vi "Main Editor UI.vi"() -> ()   [LabVIEW 2015, in "J1939 editor node.lvclass"]
doc: "This is the main view for configuration the behavior of a module in the DCAF standard editor."
uses:
  J1939 editor node.lvclass
  <vilib>/NI/Configuration Framework/Node/NodeRef.ctl
  <vilib>/NI/Configuration Framework/Node/NISE_CEF_Node.lvclass
  <vilib>/NI/AMC/Message Queue.ctl
  <vilib>/NI/AMC/Message.ctl
  <vilib>/NI/Tools/Keyed Array/KeyedArray.ctl
  <vilib>/NI/Configuration Framework/Node/UserEventRef.ctl
  <vilib>/NI/Configuration Framework/Controls/EventCluster.ctl
  <vilib>/NI/DCAF UI Toolkit/Controls/Configure.ctl
  <vilib>/NI/DCAF UI Toolkit/Controls/Add.ctl
  <vilib>/NI/DCAF UI Toolkit/Controls/Remove.ctl
  <vilib>/NI/Configuration Framework/Node/StopEvent.ctl
  <vilib>/NI/Configuration Framework/Node/RefreshUIEvent.ctl
  <vilib>/NI/Configuration Framework/Node/CacheState.ctl
  <vilib>/NI/Configuration Framework/Node/NodeChangeEvent.ctl
  <vilib>/NI/Tag Bus/tag/Data Type.ctl
  Permissions Enum.ctl
  <vilib>/NI/DCAF/Tag Editor Core/Table API/Available Tag Menu/channel action event.ctl
  <vilib>/NI/DCAF/Tag Editor Core/Table API/Available Tag Menu/dialog output action.ctl
  <vilib>/NI/Tag Bus Module Framework/channel/TBM channel.lvclass
  <vilib>/NI/Tag Bus/tag/tag descriptor.lvclass
  <vilib>/NI/DCAF/Tag Editor Core/Table API/Table Manager/Call Back Ref Type Def.ctl
  <vilib>/NI/DCAF/Tag Editor Core/Configuration Editor/Classes/Engine Parent/Engine Parent Editor Node.lvclass
  <vilib>/NI/DCAF/Tag Editor Core/Configuration Editor/Classes/Module editor node/module editor node.lvclass
  module/configuration/XNET Settings.ctl
  <vilib>/NI/DCAF/Tag Editor Core/Table API/Table Manager/references.ctl
  <vilib>/Utility/miscctls.llb/LVPositionTypeDef.ctl
  <vilib>/NI/DCAF/Tag Editor Core/Table API/Listbox/Multi Column Listbox.lvclass
  <vilib>/NI/Configuration Framework/NISE_CEF_TreeControl.lvlib
  <vilib>/NI/Tools/Keyed Array/Tools_KeyedArray.lvlib
  <vilib>/NI/AMC/AMC.lvlib
  <vilib>/NI/DCAF/Tag Editor Core/Table API/Table Manager.lvlib
  <vilib>/NI/DCAF/Tag Editor Core/Table API/Table Manager/Table Manager.lvclass
  <vilib>/NI/DCAF UI Toolkit/Controls/DCAF UI Elements.lvlib
  module/configuration/J1939 configuration.lvclass
panel:
  in  "user event out":refnum<user-event>
  in  "Permissions":T1
  in  "data type":T2
  in  "node change":T3
  in  "cache state":T4
  in  "refresh UI":T5
  in  "stop event":T6
  in  "Tab Control":enum32{"Channels", "XNET Settings"}(tab)
  in  "Remove Button":T7
  in  "Add Button":T8
  in  "Table":i32(listbox)
  in  "settings":T9
  in  "XNET Settings":T10={"Select Interface"="CAN2", "Claim By Adress"=FALSE, "Node Address"=1, "Node Name"=1}
  in  "user event":T11
  in  "main queue":T12
  in  "node ref":T13
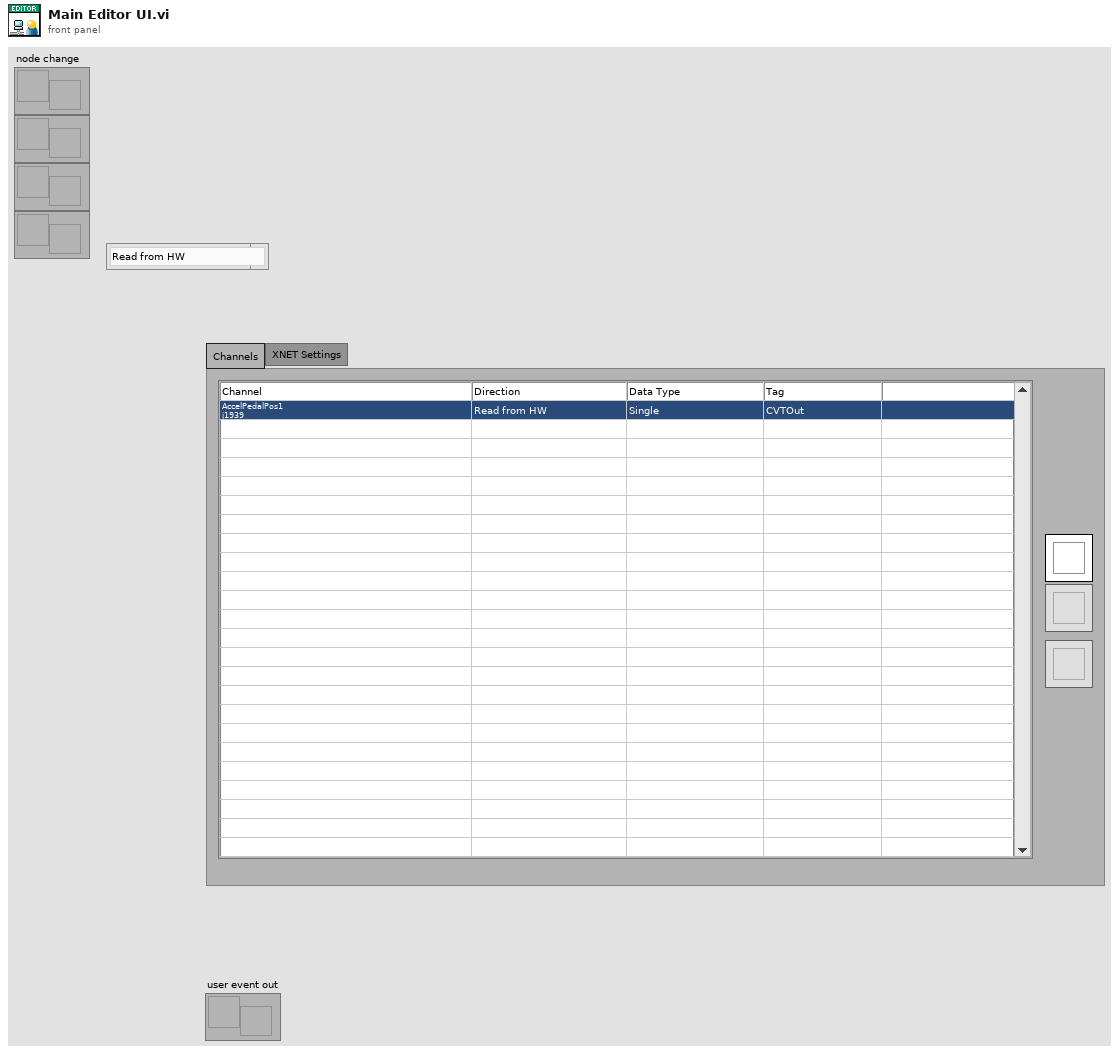
[diagram p1: front panel]
types:
  T1 = typedef "J1939 editor node.lvclass/Permissions Enum.ctl" = enum16{"Read from HW", "Write to HW"}
  T2 = typedef "tag bus.lvlib/tag descriptor.lvclass/Data Type.ctl" = enum16{"Double", "Single", "I64", "I32", "I16", "I8", "U64", "U32", "U16", "U8", "Boolean", "String", "Array of Double", "Array of Single", "Array of I64", "Array of I32", "Array of I16", "Array of I8", "Array of U64", "Array of U32", "Array of U16", "Array of U8", "Array of Boolean", "Array of String"}
  T3 = typedef "NISE_CEF_Node.lvclass/NodeChangeEvent.ctl" = refnum<user-event>
  T4 = typedef "NISE_CEF_Node.lvclass/CacheState.ctl" = refnum<user-event>
  T5 = typedef "NISE_CEF_Node.lvclass/RefreshUIEvent.ctl" = refnum<user-event>
  T6 = typedef "NISE_CEF_Node.lvclass/StopEvent.ctl" = refnum<user-event>
  T7 = typedef "DCAF UI Elements.lvlib/Remove.ctl" = bool
  T8 = typedef "DCAF UI Elements.lvlib/Add.ctl" = bool
  T9 = typedef "DCAF UI Elements.lvlib/Configure.ctl" = bool
  T10 = typedef "J1939 configuration.lvclass/XNET Settings.ctl" = cluster{"Select Interface":refnum<k21>, "Claim By Adress":bool, "Node Address":u8, "Node Name":u64}
  T11 = typedef "NISE_CEF_Node.lvclass/UserEventRef.ctl" = refnum<user-event>
  T12 = typedef "AMC.lvlib/Message Queue.ctl" = refnum<queue>
  T13 = typedef "NISE_CEF_Node.lvclass/NodeRef.ctl" = refnum<data-value>
  T14 = typedef "Table Manager.lvlib/Table Manager.lvclass/references.ctl" = cluster{"stop event":T6, "refresh UI":T5, "cache state":T4, "node change":T3, "user event out":refnum<user-event>, "main queue":T12, "user event":T11}
  T15 = typedef "LVPositionTypeDef.ctl" = cluster{"Left":i32, "Top":i32}
  T16 = typedef "Table Manager.lvlib/Table Manager.lvclass/object ref.ctl" = cluster{"engine":refnum<data-value>, "Node Ref":refnum<data-value>}
  T17 = typedef "Table Manager.lvlib/Column.lvclass/Column Descriptor.ctl" = cluster{"name":string, "caption":string, "Column Type":T18, "Params":string, "AutoSizeMode":i32, "FillWeight":sgl, "MinWidth":u32, "tooltip":string, "Enum Reference":refnum<vi>, "Channel suffix":string, "Read Only":bool, "Call Back VI":T19, "DT Dependency":i32, "name dependency":i32, "data type":T2, "Custom Column":refnum<class "Column.lvclass">}
  T18 = typedef "Table Manager.lvlib/Column.lvclass/Column Type.ctl" = enum16{"String", "Mapping", "Enum", "Custom"}
  T19 = typedef "Table Manager.lvlib/Table Manager.lvclass/Call Back Ref Type Def.ctl" = refnum<vi>
  T20 = typedef "Table Manager.lvlib/Table Manager.lvclass/Table Events.ctl" = cluster{"Menu Selection":refnum<user-event>}
  T21 = enum8{"Enabled", "Disabled", "Disabled and Grayed Out"}
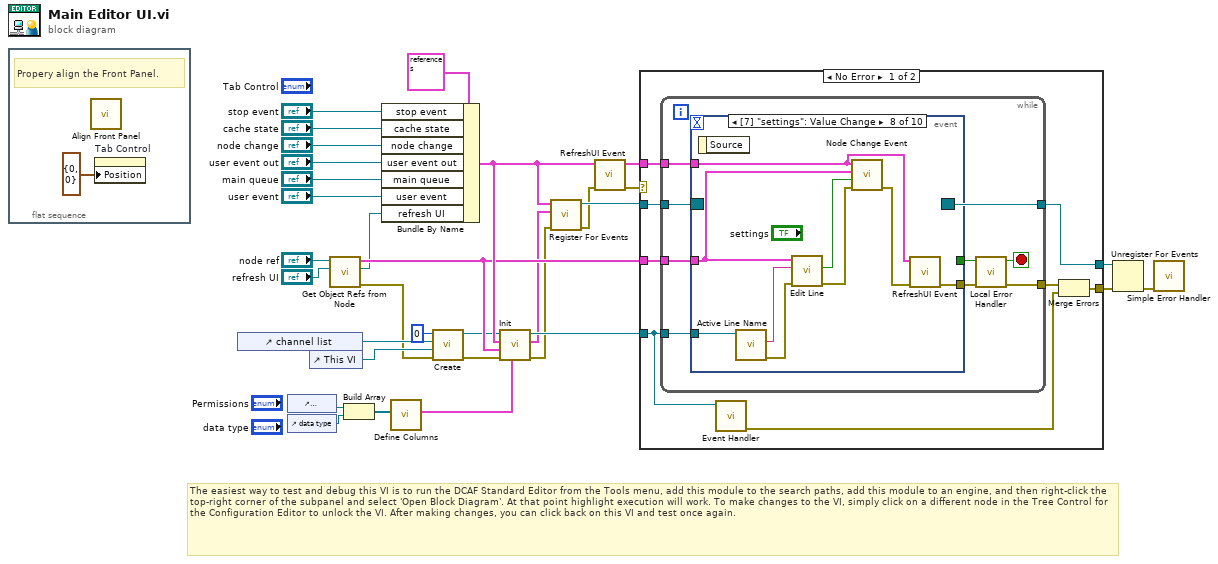
[diagram p0: block diagram]
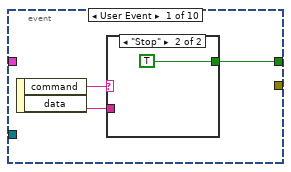
[diagram p2: hidden frame]
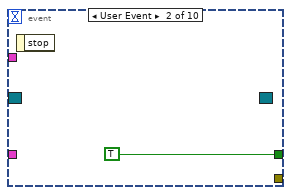
[diagram p4: hidden frame]
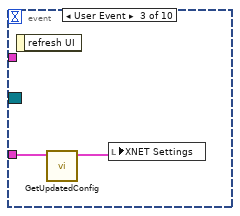
[diagram p5: hidden frame]
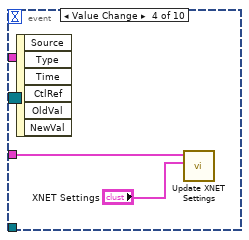
[diagram p6: hidden frame]
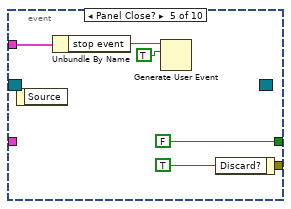
[diagram p7: hidden frame]
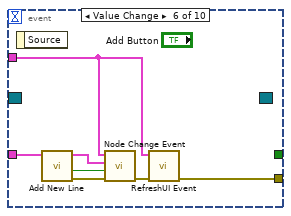
[diagram p8: hidden frame]
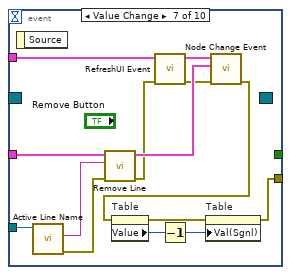
[diagram p9: hidden frame]
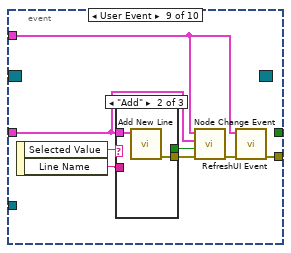
[diagram p10: hidden frame]
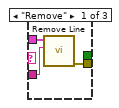
[diagram p11: hidden frame]
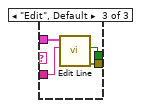
[diagram p12: hidden frame]
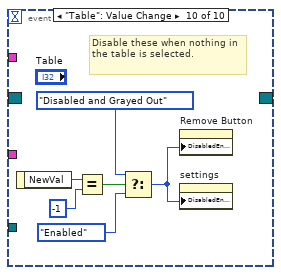
[diagram p13: hidden frame]
diagram:
  # "The easiest way to test and debug this VI is to run the DCAF Standard Editor from the Tools menu, add this module to the search paths, add this module to an engine, and then right-click the top-right corner of the subpanel and select 'Open Block Diagram'. At that point highlight execution will work. To make changes to the VI, simply click on a different node in the Tree Control for the Configuration Editor to unlock the VI. After making changes, you can click back on this VI and test once again."
  n1 = flat-sequence {
    frame #0 {
      # "Propery align the Front Panel."
      n2 = call <vilib>:"Align Front Panel.vi"() -> ()  [unwired: 10 in, 2 out]
      n3 = property on="Tab Control" class="TabCtl (strict)"("Position"=T15 {"Left"=0, "Top"=0}) -> ()  [unwired: 2 in, 2 out]
    }
  }
  n4 = control-ref of="channel list"() -> (w8:refnum<vi>)
  n5 = control-ref of="Permissions"() -> (w18:refnum<vi>)
  n6 = control-ref of="data type"() -> (w17:refnum<vi>)
  n7 = control-ref of="This VI"() -> (w6:refnum<vi>)
  n8 = call "Get Object Refs from Node.vi"("Refresh UI"="refresh UI", "Data Value Reference in"="node ref") -> ("error out"=w3:errorcluster, "Refresh UI out"=w1:T5, "References"=w15:T16)  [unwired: 7 in]
  n9 = Build Array(w18, w17) -> (w16:refnum<vi>[])
  n10 = Bundle By Name(cluster=T14 {"stop event"=refnum, "refresh UI"=refnum, "cache state"=refnum, "node change"=refnum, "user event out"=refnum, "main queue"=refnum, "user event"=refnum} ("References"), "stop event"="stop event", "cache state"="cache state", "node change"="node change", "user event out"="user event out", "main queue"="main queue", "user event"="user event", "refresh UI"=w1) -> (w19:T14)
  n11 = call "Define Columns.vi"("Enum Array"=w16) -> ("Column Definition"=w21:T17[])  [unwired: 10 in]
  n12 = call <vilib>:"Create.vi"("error in (no error)"=w3, "Top VI"=w6, "Listbox"=w8, "Index"=0) -> ("error out"=w4:errorcluster, "reference out"=w5:refnum<class "Multi Column Listbox.lvclass">)  [unwired: 6 in]
  n13 = call-dynamic "Init.vi"("Column Descriptors"=w21, "error in (no error)"=w4, "Node object refs"=w15, "Event References"=w19, "Multi Column Listbox in"=w5) -> ("error out"=w10:errorcluster, "Table Events"=w9:T20, "Multi Column Listbox out"=w14:refnum<class "Multi Column Listbox.lvclass">)  [unwired: 4 in]
  n14 = call "Register For Events.vi"("error in"=w10, "Table Events"=w9, "References"=w19) -> ("error out"=w12:errorcluster, "Event Registration Refnum"=w22:refnum<event-registration>)  [unwired: 7 in]
  n15 = call "RefreshUI Event.vi"("error in (no error)"=w12, "References in"=w19) -> ("error out"=w11:errorcluster, "References out"=w20:T14)  [unwired: 8 in]
  n16 = case shown="No Error" w11 {
    selector: w11 -> [_ w117]
    tunnel: w22 -> [w41 w116]
    tunnel: [w40 w116] -> w32
    tunnel: [w34 w117] -> w31
    tunnel: w20 -> [w39 _]
    tunnel: w15 -> [w38 _]
    tunnel: w14 -> [w37 _]
    frame No Error {
      n17 = while {
        tunnel: w41 -> [w50]
        tunnel: [w49] -> w40
        tunnel: [w46] -> w35
        tunnel: w39 -> [w44]
        tunnel: w38 -> [w43]
        tunnel: w37 -> [w42]
        stop <- w48 stop-if-true
        n18 = event shown="[7] \"settings\": Value Change" {
          selector: w50 -> [_ _ _ _ _ _ _ _ _ _]
          dyn-events: [_ _ _ _ _ _ _ _ _ _] -> w49
          timeout: _ -> [_ _ _ _ _ _ _ _ _ _]
          tunnel: [w53 TRUE _ _ FALSE _ _ _ _ _] -> w47
          tunnel: [_ _ _ _ _ w65 w72 w86 w98 _] -> w45
          tunnel: w44 -> [_ _ _ _ w61 w69 w83 w84 w94 _]
          tunnel: w43 -> [_ _ w57 w59 _ w70 w82 w90 w95 _]
          tunnel: w42 -> [_ _ _ _ _ _ w78 w91 _ _]
          event User Event {
            n19 = event-data() -> ("command"=w52:string, "data"=w51:string)  [unwired: 1 in]
            n20 = case shown="\"Stop\"" w52 {
              tunnel: [_ TRUE] -> w53
              tunnel: w51 -> [_ _]
              frame Default {
              }
              frame "Stop" {
              }
            }
          }
          event User Event {
            n21 = event-data() -> ()  [unwired: 1 in, 1 out]
          }
          event User Event {
            n22 = event-data() -> ()  [unwired: 1 in, 1 out]
            n23 = call "GetUpdatedConfig.vi"("References"=w57) -> ("XNET Settings"=w56:T10)  [unwired: 10 in]
            n24 = local write "XNET Settings"(w56) -> ()
          }
          event Value Change {
            n25 = event-data() -> ()  [unwired: 1 in, 6 out]
            n26 = call "Update XNET Settings.vi"("XNET Settings"="XNET Settings", "References"=w59) -> ()  [unwired: 10 in]
          }
          event Panel Close? {
            n27 = event-data() -> ()  [unwired: 1 in, 1 out]
            n28 = Unbundle By Name(w61) -> ("stop event"=w60:T6)
            n29 = Generate User Event(user event=w60, event data cluster=TRUE ("event data")) -> ()  [unwired: 2 in, 2 out]
            n30 = event-data("Discard?"=TRUE) -> ()  [unwired: 1 in, 1 out]
          }
          event Value Change {
            n31 = event-data() -> ()  [unwired: 1 in, 1 out]
            n32 = call "Add New Line.vi"("objects"=w70) -> ("error out"=w68:errorcluster, "success"=w66:bool)  [unwired: 8 in, 1 out]
            n33 = call "Node Change Event.vi"("error in (no error)"=w68, "Send (T)"=w66, "objects"=w70, "References in"=w69) -> ("error out"=w67:errorcluster)  [unwired: 7 in]
            n34 = call "RefreshUI Event.vi"("error in (no error)"=w67, "References in"=w69) -> ("error out"=w65:errorcluster)  [unwired: 8 in, 1 out]
          }
          event Value Change {
            n35 = event-data() -> ()  [unwired: 1 in, 1 out]
            n36 = call-dynamic "Active Line Name.vi"("Multi Column Listbox in"=w78) -> ("error out"=w76:errorcluster, "Active Line Name"=w77:string)  [unwired: 8 in, 1 out]
            n37 = call "Remove Line.vi"("error in"=w76, "Active Line Name"=w77, "Objects"=w82) -> ("error out"=w79:errorcluster)  [unwired: 8 in]
            n38 = call "RefreshUI Event.vi"("error in (no error)"=w79, "References in"=w83) -> ("error out"=w81:errorcluster, "References out"=w80:T14)  [unwired: 8 in]
            n39 = call "Node Change Event.vi"("error in (no error)"=w81, "objects"=w82, "References in"=w80) -> ("error out"=w73:errorcluster)  [unwired: 8 in]
            n40 = property on="Table" class="MCListbox (strict)"(error in=w73) -> (error out=w71:errorcluster, "Value"=w74:i32)  [unwired: 1 in, 1 out]
            n41 = Decrement(x=w74) -> (x-1=w75:i32)
            n42 = property on="Table" class="MCListbox (strict)"(error in=w71, "Val(Sgnl)"=w75) -> (error out=w72:errorcluster)  [unwired: 1 in, 1 out]
          }
          event Value Change {
            n43 = event-data() -> ()  [unwired: 1 in, 1 out]
            n44 = call-dynamic "Active Line Name.vi"("Multi Column Listbox in"=w91) -> ("error out"=w88:errorcluster, "Active Line Name"=w89:string)  [unwired: 8 in, 1 out]
            n45 = call "Edit Line.vi"("error in"=w88, "Line Name"=w89, "References"=w90) -> ("error out"=w92:errorcluster, "change?"=w87:bool)  [unwired: 7 in]
            n46 = call "Node Change Event.vi"("error in (no error)"=w92, "Send (T)"=w87, "objects"=w90, "References in"=w84) -> ("error out"=w85:errorcluster)  [unwired: 7 in]
            n47 = call "RefreshUI Event.vi"("error in (no error)"=w85, "References in"=w84) -> ("error out"=w86:errorcluster)  [unwired: 8 in, 1 out]
          }
          event User Event {
            n48 = event-data() -> ("Selected Value"=w100:string, "Line Name"=w97:string)  [unwired: 1 in]
            n49 = case shown="\"Add\"" w100 {
              tunnel: w97 -> [w103 _ w109]
              tunnel: w95 -> [w102 w105 w108]
              tunnel: [w101 w104 w107] -> w96
              tunnel: [_ _ w106] -> w93
              frame "Remove" {
                n50 = call "Remove Line.vi"("Active Line Name"=w103, "Objects"=w102) -> ("error out"=w101:errorcluster)  [unwired: 9 in]
              }
              frame "Add" {
                n51 = call "Add New Line.vi"("objects"=w105) -> ("error out"=w104:errorcluster)  [unwired: 8 in, 2 out]
              }
              frame "Edit", Default {
                n52 = call "Edit Line.vi"("Line Name"=w109, "References"=w108) -> ("error out"=w107:errorcluster, "change?"=w106:bool)  [unwired: 8 in]
              }
            }
            n53 = call "Node Change Event.vi"("error in (no error)"=w96, "Send (T)"=w93, "objects"=w95, "References in"=w94) -> ("error out"=w99:errorcluster)  [unwired: 7 in]
            n54 = call "RefreshUI Event.vi"("error in (no error)"=w99, "References in"=w94) -> ("error out"=w98:errorcluster)  [unwired: 8 in, 1 out]
          }
          event "Table": Value Change {
            # "Disable these when nothing in the table is selected."
            n55 = event-data() -> ("NewVal"=w115:i32)  [unwired: 1 in]
            n56 = Equal?(x=w115, y=-1) -> (x = y?=w113:bool)
            n57 = Select(t=T21."Disabled and Grayed Out" ("Disabled"), s=w113, f=T21."Enabled") -> (s? t:f=w111:T21)
            n58 = property on="Remove Button" class="Bool"("DisabledEnum"=w111) -> ()  [unwired: 2 in, 2 out]
            n59 = property on="settings" class="Bool"("DisabledEnum"=w111) -> ()  [unwired: 2 in, 2 out]
          }
        }
        n60 = call "Local Error Handler.vi"("error in"=w45, "Stop in"=w47) -> ("error out"=w46:errorcluster, "Stop out"=w48:bool)  [unwired: 8 in]
      }
      n61 = call-dynamic "Event Handler.vi"("Listbox in"=w37) -> ("error out"=w36:errorcluster)  [unwired: 9 in, 1 out]
      n62 = Merge Errors(w35, w36) -> (w34:errorcluster)
    }
    frame Error {
    }
  }
  n63 = Unregister For Events(event registration refnum=w32, error in=w31) -> (error out=w30:errorcluster)
  n64 = call <vilib>:"Simple Error Handler.vi"("error in (no error)"=w30) -> ()  [unwired: 4 in, 5 out]
